vi "test_lab_3_3.vi"() -> ()   [LabVIEW 2025]
uses:
  <vilib>/rvi/DesktopExecutionNode/Execution/niFpgaDEN_Execute.vi
  <vilib>/rvi/interface/RandomDataEmulation/nirviRandomDataOpen.vi
  <vilib>/rvi/interface/common/niFpgaCacheSessionInfoDynamic.vi
  <vilib>/rvi/interface/common/niFpgaWaitOnOcc.vi
  <vilib>/Utility/error.llb/Error Cluster From Error Code.vi
  <vilib>/rvi/errors/niLvFpgaAdjustHostInterfaceError.vi
  <vilib>/FPGAPlugInAG/Dynamic/niLvFpga_Run_Dynamic.vi
  <vilib>/FPGAPlugInAG/Dynamic/niLvFpga_Close_Dynamic.vi
  <vilib>/rvi/DesktopExecutionNode/DesktopExecutionNode.xnode
  <vilib>/rvi/interface/nirviOpenFPGA/nirviOpenFPGA.xnode
  BartlomiejRaczynski/vi/lab3_1.vi
  <vilib>/rvi/interface/nirviMethod/nirviMethod.xnode
  <vilib>/rvi/interface/nirviReadWriteControl/nirviReadWriteControl.xnode
  <vilib>/rvi/interface/nirviCloseFPGA/nirviCloseFPGA.xnode
  <vilib>/FPGAPlugInAG/Dynamic/niLvFpga_ReadFifo_Dynamic.vi
  <vilib>/rvi/errors/niLvFpgaMergeErrorWithErrorCode.vi
  <vilib>/FPGAPlugInAG/Dynamic/niLvFpga_ConfigureFifo_Dynamic.vi
  NiFpgaLv.dll
  <vilib>/rvi/interface/Simulation/niFpgaSimulationCallBeginRW.vi
panel:
  out "error out":errorcluster
  in  "Shake forward":bool
  in  "Shake left":bool
  out "Elements Remaining":u32
  in  "Stop":bool
  out "Waveform Graph":i16[](graph)
  in  "Treshold":i16
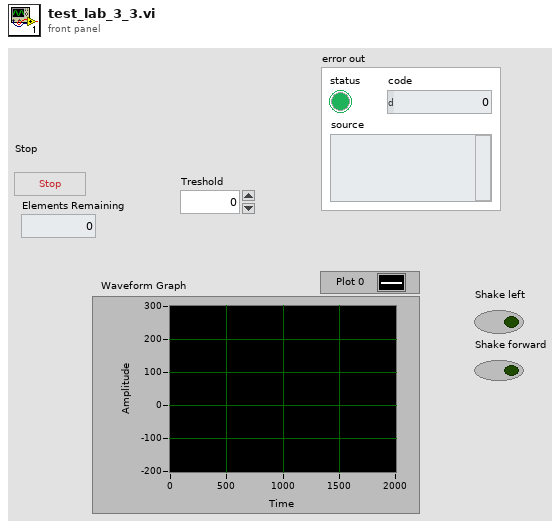
[diagram p1: front panel]
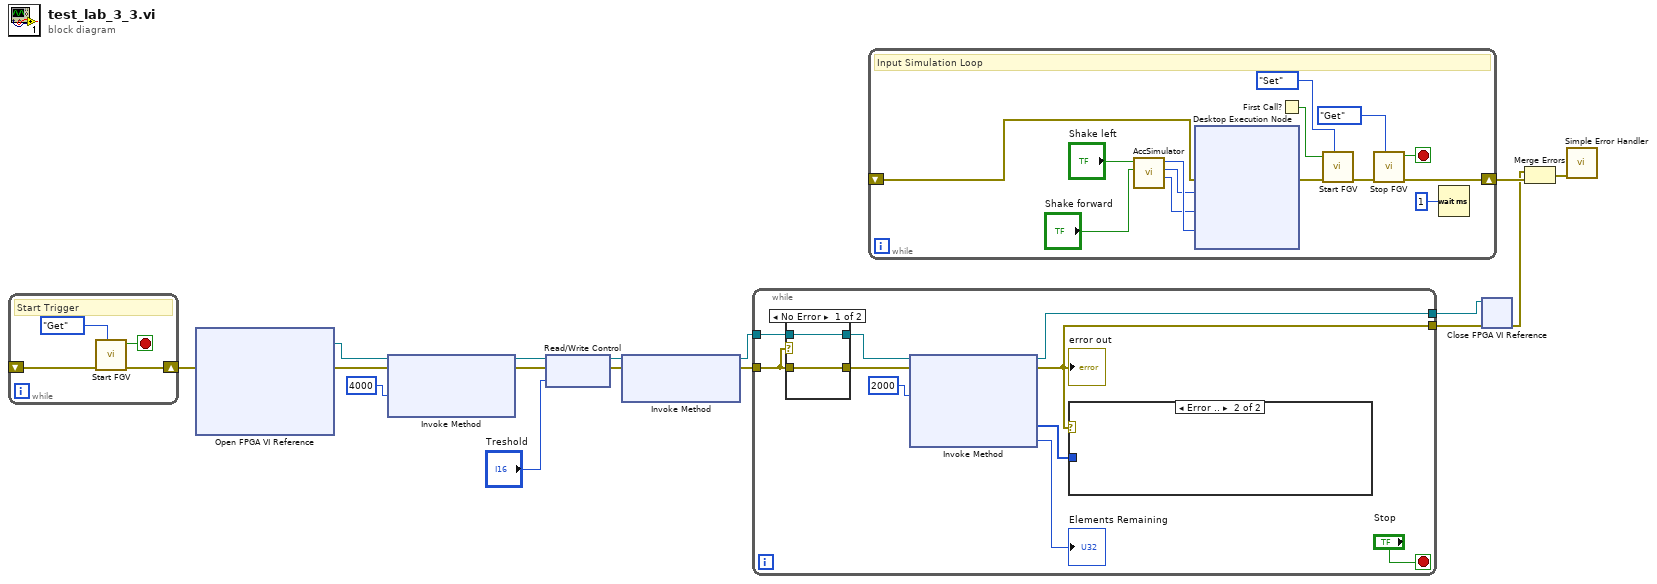
[diagram p0: block diagram]
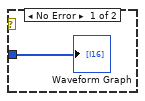
[diagram p2: hidden frame]
diagram:
  n1 = while {
    shift-right: [w20] -> w7
    shift-left: _ -> [w18]
    stop <- w19 stop-if-true
    # "Start Trigger"
    n2 = call "Start FGV.vi"("Mode"=enum16{"Set", "Get"}."Get", "Error In"=w18) -> ("Error Out"=w20:errorcluster, "Get Value"=w19:bool)  [unwired: 8 in]
  }
  n3 = xnode "Open FPGA VI Reference"("error in"=w7) -> ("FPGA VI Reference Out"=w12:refnum<k20>, "error out"=w11:errorcluster)  [unwired: 1 in]
  n4 = xnode "Invoke Method"("FPGA VI Reference In"=w12, "error in"=w11, "Requested Depth"=u32 4000) -> ("FPGA VI Reference Out"=w13:refnum<k20>, "error out"=w14:errorcluster)  [unwired: 1 out]
  n5 = xnode "Read/Write Control"("FPGA VI Reference In"=w13, "error in"=w14, "Treshold"="Treshold") -> ("FPGA VI Reference Out"=w6:refnum<k20>, "error out"=w5:errorcluster)
  n6 = xnode "Invoke Method"("FPGA VI Reference In"=w6, "error in"=w5) -> ("FPGA VI Reference Out"=w4:refnum<k20>, "error out"=w3:errorcluster)  [unwired: 1 in]
  n7 = while {
    tunnel: w4 -> [w26]
    tunnel: w3 -> [w25]
    tunnel: [w23] -> w9
    tunnel: [w21] -> w8
    stop <- "Stop" stop-if-true
    n8 = case shown="No Error" w25 {
      tunnel: w26 -> [w33 w35]
      tunnel: [w33 w35] -> w30
      tunnel: w25 -> [w32 w34]
      tunnel: [w32 w34] -> w29
      frame No Error {
      }
      frame Error {
      }
    }
    n9 = xnode "Invoke Method"("FPGA VI Reference In"=w30, "error in"=w29, "Number of Elements"=u32 2000) -> ("FPGA VI Reference Out"=w23:refnum<k20>, "error out"=w21:errorcluster, "Data"=w22:i16[], "Elements Remaining"=→"Elements Remaining":u32)  [unwired: 1 in]
    "error out" <- w21
    n10 = case shown="Error .." w21 {
      tunnel: w22 -> [w31 _]
      frame No Error {
        "Waveform Graph" <- w31
      }
      frame Error {
      }
    }
  }
  n11 = while {
    shift-right: [w44] -> w16
    shift-left: _ -> [w41]
    stop <- w45 stop-if-true
    # "Input Simulation Loop"
    n12 = call "AccSimulator.vi"("Shake forward"="Shake forward", "Shake left"="Shake left") -> ("Acc Y"=w38:i16, "Acc X"=w39:i16, "Acc Z"=w40:i16)  [unwired: 7 in]
    n13 = xnode "Desktop Execution Node"("Error In"=w41, "AccelerationX"=w39, "AccelerationY"=w38, "AccelerationZ"=w40) -> ("Error Out"=w42:errorcluster)
    n14 = First Call?() -> (First Call?: T/F=w49:bool)
    n15 = call "Start FGV.vi"("Mode"=enum16{"Set", "Get"}."Set", "Error In"=w42, "Set Value"=w49) -> ("Error Out"=w47:errorcluster)  [unwired: 7 in, 1 out]
    n16 = call "Stop FGV.vi"("Mode"=enum16{"Set", "Get"}."Get", "Error In"=w47) -> ("Error Out"=w44:errorcluster, "Get Value"=w45:bool)  [unwired: 8 in]
    n17 = Wait (ms)(milliseconds to wait=u32 1 ("millisecond multiple")) -> ()  [unwired: 1 out]
  }
  n18 = xnode "Close FPGA VI Reference"("FPGA VI Reference In"=w9, "error in"=w8) -> ("error out"=w1:errorcluster)
  n19 = Merge Errors(w1, w16) -> (w15:errorcluster)
  n20 = call <vilib>:"Simple Error Handler.vi"("error in (no error)"=w15) -> ()  [unwired: 4 in, 5 out]
